vi "AnyBuilderBuild.vi"(8 "error in":errorcluster, 10 "Message Type":string, 11 "Builder Ref":T2) -> (0 "error out":errorcluster, 3 "Any":T1)   [LabVIEW 2019, in "grpc-lvsupport.lvlib"]
uses:
  grpc-lvsupport.lvlib
  Shared/grpcId.ctl
  Shared/Any.ctl
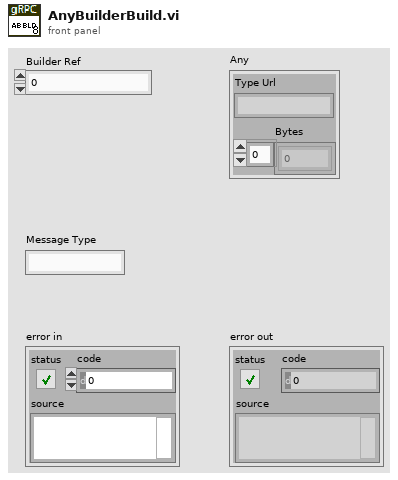
[diagram p1: front panel]
types:
  T1 = typedef "grpc-lvsupport.lvlib/Any.ctl" = cluster{"Type Url":string, "Bytes":u8[]}
  T2 = typedef "grpc-lvsupport.lvlib/grpcId.ctl" = u64
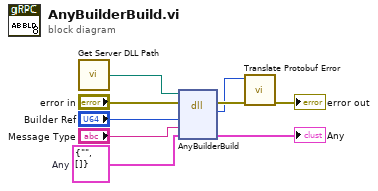
[diagram p0: block diagram]
diagram:
  w4 = T1 {"Type Url"="", "Bytes"=[]}  # Any
  n1 = call "Get Server DLL Path.vi"() -> ("Server dll path"=w7:path)
  n2 = dll-call lib="?" fn="AnyBuilderBuild"(path in=w7, error in="error in", "builderId"="Builder Ref", "messageType"="Message Type", "any"=w4) -> (error out=w8:errorcluster, "return type"=w1:i32, "any"=→"Any":T1)  [unwired: 3 in, 1 out]
  n3 = call "Translate Protobuf Error.vi"("error in"=w8, "Error Code"=w1) -> ("error out"=→"error out":errorcluster)  [unwired: 9 in]
